vi "I2C M5Stack Ultrasonic.vi"() -> ()   [LabVIEW 2020, in "CTI-Scratchpad.lvlib"]
uses:
  CTI-Scratchpad.lvlib
  CTI/Identity.ctl
  CTI/Error Reporting.ctl
  CTI/I2C Address.ctl
  CTI/GPIO Number.ctl
  CTI/I2C Number.ctl
  CTI/Session/Session.lvclass
  CTI-Peripheral/Ranging Sensor/M5Stack UltraSonic Range Sensor.lvclass
  CTI/VisaComms/VisaComms.lvclass
  CTI/CTI.lvlib
panel:
  out "Thermometer":dbl(slide) scale=0.0..4500.0
  out "Distance":dbl(graph)
  in  "Stop":bool
  out "loop":i32
  out "Identity":T1
  in  "Grove Connector":enum16{"I2C0", "I2C1"}(ring)
  out "error out":errorcluster
  in  "Port":refnum<visa-resource-name>="COM4"
  # "https://docs.m5stack.com/en/unit/Unit_Ultrasonic-I2C"
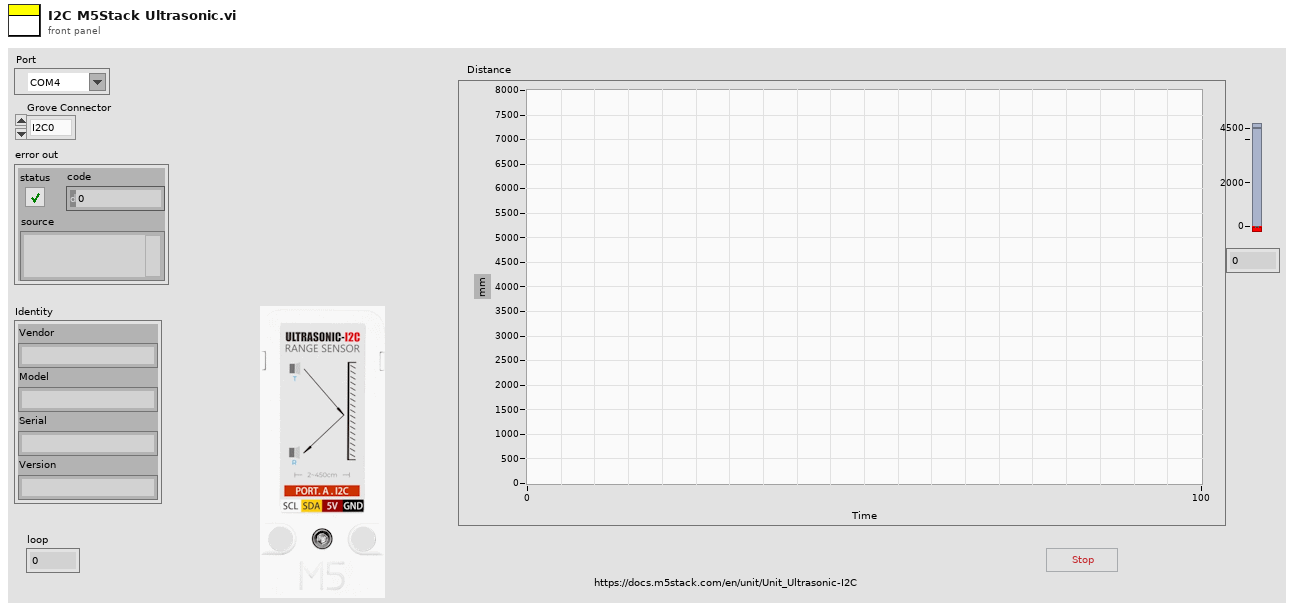
[diagram p1: front panel]
types:
  T1 = typedef "CTI.lvlib/Identity.ctl" = cluster{"Vendor":string, "Model":string, "Serial":string, "Version":string}
  T2 = typedef "CTI.lvlib/I2C Address.ctl" = u8
  T3 = typedef "CTI.lvlib/Error Reporting.ctl" = enum16{"Minimal", "Moderate", "Full"}
  T4 = typedef "CTI.lvlib/I2C Number.ctl" = i8
  T5 = typedef "CTI.lvlib/GPIO Number.ctl" = i8
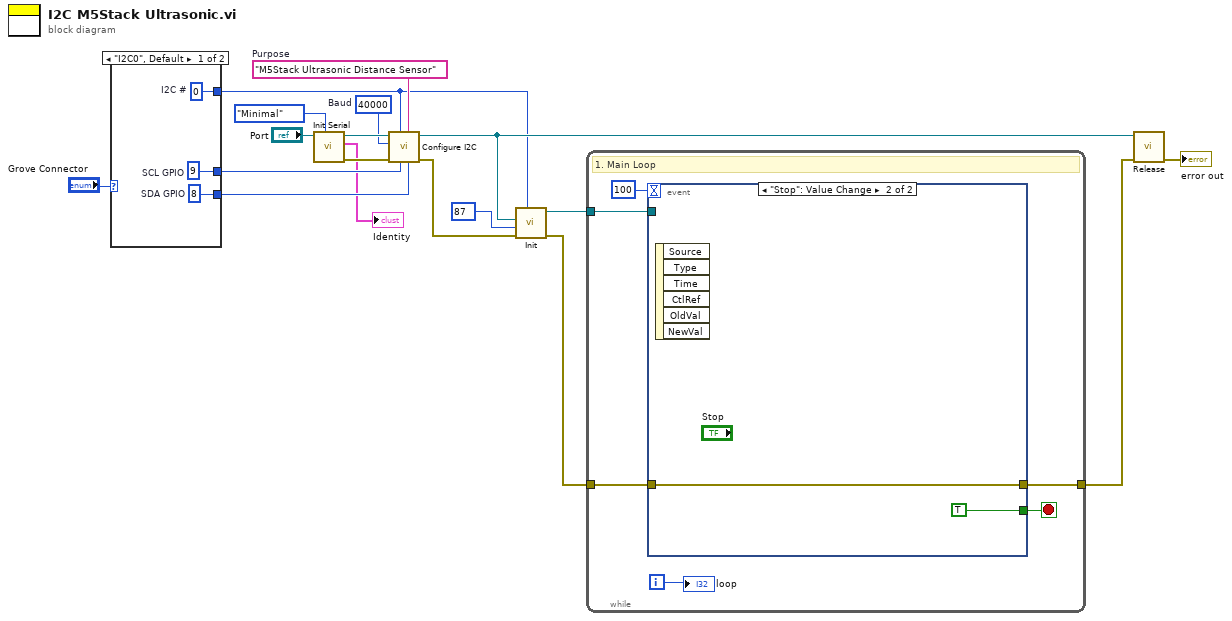
[diagram p0: block diagram]
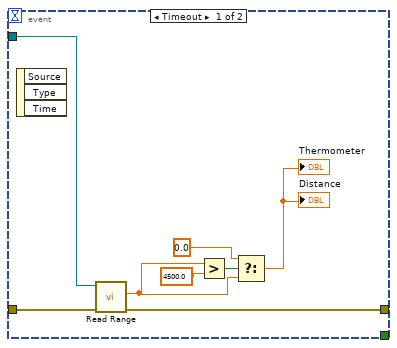
[diagram p2: hidden frame]
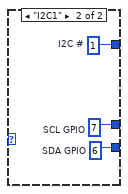
[diagram p3: hidden frame]
diagram:
  w13 = "M5Stack Ultrasonic Distance Sensor"  # Purpose
  w14 = u32 40000  # Baud
  n1 = case shown="\"I2C0\", Default" "Grove Connector" {
    tunnel: [w21 w24] -> w11
    tunnel: [w20 w23] -> w10
    tunnel: [w19 w22] -> w4
    frame "I2C0", Default {
      w19 = T4 0  # I2C #
      w20 = T5 8  # SDA GPIO
      w21 = T5 9  # SCL GPIO
    }
    frame "I2C1" {
      w22 = T4 1  # I2C #
      w23 = T5 6  # SDA GPIO
      w24 = T5 7  # SCL GPIO
    }
  }
  n2 = call "Init Serial.vi"("Error Checking (Full)"=Error_Reporting."Minimal", "VISA resource name in"="Port") -> ("error out"=w15:errorcluster, "Identity"=→"Identity":T1, "Session"=w16:refnum<class "Session.lvclass">)  [unwired: 7 in]
  n3 = call "Configure I2C.vi"("SDA GPIO"=w10, "Purpose (\"I2C\")"=w13, "SCL GPIO"=w11, "I2C #"=w4, "error in (no error)"=w15, "Baud"=w14, "Session in"=w16) -> ("error out"=w6:errorcluster, "Session out"=w5:refnum<class "Session.lvclass">)  [unwired: 3 in]
  n4 = call "Init.vi"("I2C #"=w4, "error in (no error)"=w6, "Address"=T2 87, "Session In"=w5) -> ("error out"=w3:errorcluster, "M5Stack UltraSonic Range Sensor Out"=w2:refnum<class "M5Stack UltraSonic Range Sensor.lvclass">)  [unwired: 6 in]
  n5 = while {
    tunnel: w3 -> [w29]
    tunnel: w2 -> [w30]
    tunnel: [w27] -> w8
    i -> [w28]
    stop <- w25 stop-if-true
    # "1. Main Loop"
    n6 = event shown="[1] \"Stop\": Value Change" {
      selector: _ -> [_ _]
      dyn-events: _ -> [_ _]
      timeout: 100 -> [_ _]
      tunnel: w30 -> [w36 _]
      tunnel: w29 -> [w38 w39]
      tunnel: [w37 w39] -> w27
      tunnel: [_ TRUE] -> w25
      event Timeout {
        n7 = event-data() -> ()  [unwired: 1 in, 3 out]
        n8 = call-dynamic "Read Range.vi"("error in (no error)"=w38, "M5Stack UltraSonic Range  in"=w36) -> ("error out"=w37:errorcluster, "Range"=w32:dbl)  [unwired: 7 in, 1 out]
        n9 = Greater?(x=w32, y=4500.0) -> (0:w34:bool)
        n10 = Select(t=0.0, s=w34, f=w32) -> (s? t:f=→"Distance" →"Thermometer":dbl)
      }
      event "Stop": Value Change {
        n11 = event-data() -> ()  [unwired: 1 in, 6 out]
      }
    }
    "loop" <- w28
  }
  n12 = call-dynamic "Release.vi"("error in (no error)"=w8, "Session in"=w5) -> ("error out"=→"error out":errorcluster)  [unwired: 9 in]
